vi "work1_GetOrder and Cook.vi"() -> ()   [LabVIEW 2026]
panel:
  out "Client Served":i32
  out "Order ID":i32
  in  "Numeric":i32
  in  "stop":bool
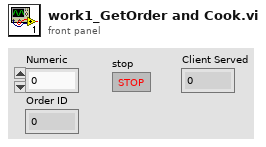
[diagram p1: front panel]
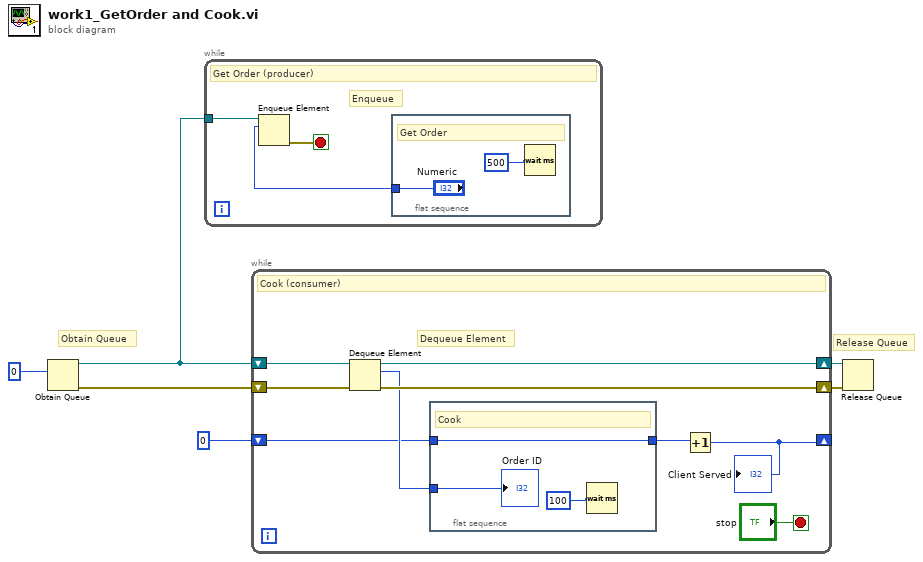
[diagram p0: block diagram]
diagram:
  # "Release Queue"
  # "Obtain Queue"
  n1 = Obtain Queue(element data type=0) -> (queue out=w3:refnum<queue>, error out=w6:errorcluster)  [unwired: 4 in, 1 out]
  n2 = while {
    tunnel: w3 -> [w9]
    stop <- w8 stop-if-true
    # "Enqueue"
    # "Get Order (producer)"
    n3 = Enqueue Element(queue=w9, element=w7) -> (error out=w8:errorcluster)  [unwired: 2 in, 2 out]
    n4 = flat-sequence {
      tunnel: ["Numeric"] -> w7
      frame #0 {
        # "Get Order"
        n5 = Wait (ms)(milliseconds to wait=u32 500) -> ()  [unwired: 1 out]
      }
    }
  }
  n6 = while {
    shift-right: [w18] -> w4
    shift-left: w6 -> [w20]
    shift-right: [w19] -> w5
    shift-left: w3 -> [w17]
    shift-right: [w12] -> _
    shift-left: 0 -> [w15]
    stop <- "stop" stop-if-true
    # "Dequeue Element"
    # "Cook (consumer)"
    n7 = Dequeue Element(queue=w17, error in (no error)=w20) -> (queue out=w19:refnum<queue>, element=w16:i32, error out=w18:errorcluster)  [unwired: 1 in, 1 out]
    n8 = flat-sequence {
      tunnel: w16 -> [w22]
      tunnel: w15 -> [w21]
      tunnel: [w21] -> w14
      frame #0 {
        # "Cook"
        n9 = Wait (ms)(milliseconds to wait=u32 100) -> ()  [unwired: 1 out]
        "Order ID" <- w22
      }
    }
    n10 = Increment(x=w14) -> (x+1=w12:i32)
    "Client Served" <- w12
  }
  n11 = Release Queue(queue=w5, error in (no error)=w4) -> ()  [unwired: 1 in, 3 out]
